vi "AlliGator Lifetime & Other Parameters Panel.vi"() -> ()   [LabVIEW 2021, in "AlliGator Lifetime & Other Parameters.lvlib"]
uses:
  AlliGator Lifetime & Other Parameters.lvlib
  AlliGator Lifetime & Other Parameters Ctrl Refnums.ctl
  Globals, Variables, Constants/AlliGator Refnums List.ctl
  Settings/AlliGator Settings List.ctl
  Graphs/XY Graph/XY Graph Event.ctl
  <vilib>/Utility/miscctls.llb/LVPoint32TypeDef.ctl
  Action Engine/AlliGator Q Element.ctl
  Action Engine/AlliGator Q Event.ctl
  Graphs/XY Graph/New Plot Information.ctl
  Graphs/Plot Scales.ctl
  Graphs/LabVIEW Plot Interpolation.ctl
  Graphs/Plot Point Style.ctl
  Graphs/XY Graph/XY Graph Mouse Click Event Data.ctl
  Graphs/XY Graph/XY Graph Refnum.ctl
  Variant/Variant to Data/Variant to Boolean.vi
  Settings/AlliGator Settings+.lvlib
  Variant/Variant to Data/Variant to Data.lvlib
  Notebook/Notebook.lvlib
  Action Engine/AlliGator Action Engine.lvlib
  GUI/GUI.lvlib
  GUI/AlliGator GUI.lvlib
  Error/Error.lvlib
  Graphs/XY Graph/XY Graph Add-Ons.lvlib
  Python Plugins API/AlliGator Python Plugins.lvlib
  Decay Analysis/Decay Processing/AlliGator Decay Processing.lvlib
  Graphs/Graphs.lvlib
  Phasor Ratio/AlliGator Phasor Ratio.lvlib
  Utilities/Utilities.lvlib
panel:
  in  "Pin Button":bool=TRUE
  out "Lifetime & Other Parameters Graph TipStrip":string caption="Lifetime Graph TipStrip"
  out "Lifetime & Other Parameters Graph":cluster{"X Array":dbl[], "Y Array":dbl[]}[](graph)
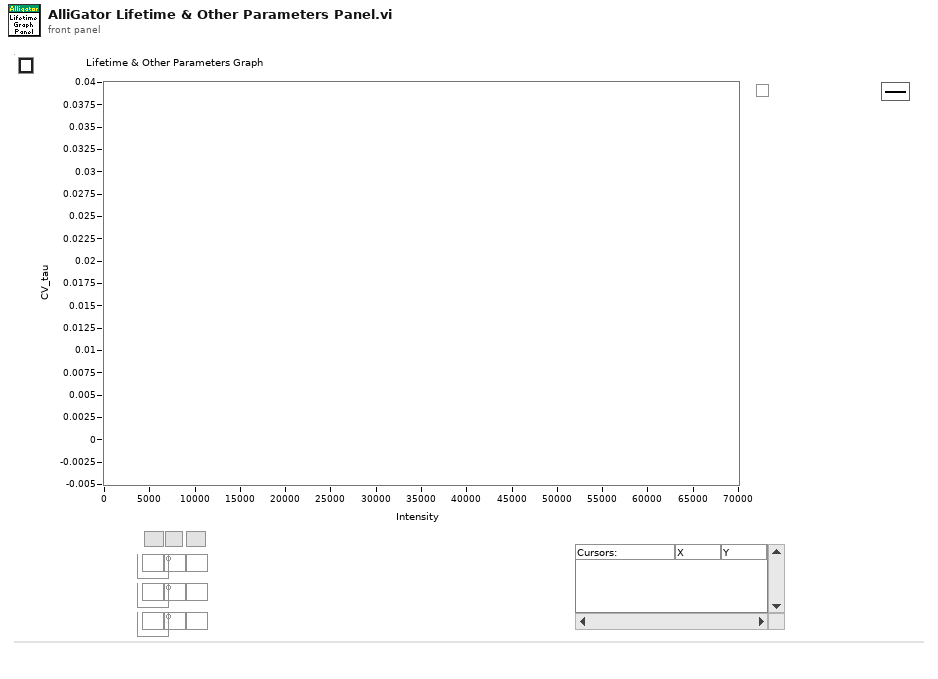
[diagram p1: front panel]
types:
  T1 = typedef "AlliGator GUI.lvlib/AlliGator Refnums List.ctl" = enum16{"---------- AlliGator Control Refnums ----------", "AlliGator Tab Control Refnum", "Dataset Ctrl Refnums", "Image Histogram Ctrl Refnums", "Intensity Time Trace Ctrl Refnums", "Decay Graph Ctrl Refnums", "Decay Statistics Graph Ctrl Refnums", "Phasor Graph Ctrl Refnums", "Phasor Ratio Graph Ctrl Refnums", "Phasor Plot Ctrl Refnums", "Lifetime & Other Parameters Ctrl Refnums", "Decay Fit Parameter Map Ctrl Refnums", "Parameter Map Ctrl Refnums", "Other AlliGator Ctrl Refnums", "---------- AlliGator Menu Refnums ----------", "AlliGator Menu", "---------- IO Device ID ----------", "Mouse ID", "Keyboard ID"}
  T2 = typedef "AlliGator Lifetime & Other Parameters.lvlib/AlliGator Lifetime & Other Parameters Ctrl Refnums.ctl" = cluster{"Lifetime Graph":refnum<vi>}
  T3 = cluster{"Event Registration Refnum":refnum<event-registration>, "Event Registration Refnum":refnum<event-registration>}
  T4 = typedef "AlliGator Settings+.lvlib/AlliGator Settings List.ctl" = enum16{"GUI:Visible Settings Tab", "GUI:Last Run Version", "Source Image:Use Image Histogram for Contrast", "Source Image:Low Count Pixels Rejection Options", "Source Image:High Count Pixels Rejection Options", "Source Image:Use Image Brightness", "Source Image:Blend Overlay with Image Background", "Source Image:Use Fixed ROI Diameter", "Source Image:ROI Diameter", "Source Image:ROI Center Color", "Source Image:Peak Threshold", "Source Image:Intensity Threshold", "Source Image:Image Binning Options", "Source Image:Image Smoothing Options", "Source Image:Image Histogram Active", "Source Image:Invert Binary Mask", "Source Image:Hot Pixel Removal", "Source Image:Overlay Analyzed ROI Center", "Source Image:Auto-Adjust Contrast", "Source Image:Histogram Lower Percentile", "Source Image:Histogram Upper Percentile", "Source Image:Lock ROI with Maps", "Source Image:Save Source Image", "Source Image:Scale Bar Options", "Source Image:Image Resolution (Pixel Size)", "Source Image:Flatfield Correction", "Source Image:Show Dead Left Columns Correction", "Source Image:Dead Left Columns Correction", "Source Image:Image Pre-Processing Operations Order", "Source Image:Overlay ROI Median", "Source Image:Median Overlay Color", "Data Information:Gate Width", "Data Information:Nanotime Gate Separation", "Data Information:Macrotime Gate Separation", "Data Information:Gate Step", "Data Information:# Gates", "Data Information:Gate Image Exposure", "Data Information:Gate Image Integration", "Data Information:Gates to Skip", "Data Information:Gates to Keep", "Data Information:Define Gates to", "Data Information:Channel Name", "Data Information:Available Channel Names", "Data Information:Channel Arithmetic", "Data Information:Background File Subtraction", "Data Information:Background File", "Data Information:Background Scaling Factor", "Data Information:Background Pile-up Correction", "Data Information:Background Pixel Well Capacity", "Data Information:Laser Period", "Data Information:SYNC Period", "Data Information:Pile-up Correction", "Data Information:Pixel Well Capacity", "Data Information:Dataset Scaling Factor", "Fluorescence Decay_Decay Pre-Processing:Reverse Gates", "Fluorescence Decay_Decay Pre-Processing:Verbose Decay Pre-Processing", "Fluorescence Decay_Decay Pre-Processing:Use Decay Pre-Processing", "Fluorescence Decay_Decay Pre-Processing:Background Subtraction", "Fluorescence Decay_Decay Pre-Processing:Background Definition Range", "Fluorescence Decay_Decay Pre-Processing:Baseline Subtraction Method", "Fluorescence Decay_Decay Pre-Processing:Decay Pre-Processing Operations Order", "Fluorescence Decay_Decay Pre-Processing:Smoothing Parameter", "Fluorescence Decay_Decay Pre-Processing:Shift Decay", "Fluorescence Decay_Decay Pre-Processing:Decay Shift Parameters", "Fluorescence Decay_Decay Pre-Processing:Fold Decay", "Fluorescence Decay_Decay Pre-Processing:# Folds", "Fluorescence Decay_Decay Pre-Processing:1-Normalize Decay", "Fluorescence Decay_Decay Pre-Processing:[0-1]-Normalize Decay", "Fluorescence Decay_Decay Pre-Processing:Smoothen Decay", "Fluorescence Decay_Decay Pre-Processing:Extrapolate Decay", "Fluorescence Decay_Decay Pre-Processing:Use Periodicity", "Fluorescence Decay_Decay Pre-Processing:Use Cursors", "Fluorescence Decay_Decay Pre-Processing:Tail Fraction", "Fluorescence Decay_Decay Pre-Processing:Head Fraction", "Fluorescence Decay_Decay Pre-Processing:Additional Points", "Fluorescence Decay_Decay Pre-Processing:Straighten Decay", "Fluorescence Decay_Decay Pre-Processing:Constant Background", "Fluorescence Decay_Decay Pre-Processing:Pixel-Normalize Decay", "Fluorescence Decay_Advanced Analysis:Extract IRF instead of Decay", "Fluorescence Decay_Advanced Analysis:IRF Extraction Options", "Fluorescence Decay_Advanced Analysis:IRF Optimization Options", "Fluorescence Decay_Advanced Analysis:Square Pulse Options", "Fluorescence Decay_Advanced Analysis:IRF Order", "Fluorescence Decay_Advanced Analysis:IRF Time Constants", "Fluorescence Decay_Advanced Analysis:Wavelet Analysis Options", "Fluorescence Decay_Advanced Analysis:Average Lifetime Options", "Fluorescence Decay_Fit Options:Fit Options", "Fluorescence Decay_Fit Options:Use Legacy Fitting Approach", "Fluorescence Decay_Fit Options:Use Data Information Laser Period", "Fluorescence Decay_Fit Parameters:Displayed Fit Parameters", "Fluorescence Decay_Fit Parameters:Fit Parameter Constraints", "Fluorescence Decay_Fit Parameters:Export Tabulated Results", "Fluorescence Decay_Fit Parameters:MLE Baseline Offset Type", "Fluorescence Decay_Fit Parameters:MLE Baseline Offset", "Fluorescence Decay_Fit Parameters:Guess Parameter Names", "Fluorescence Decay_Fit Parameters:Guess Parameter Values", "Fluorescence Decay_Fit Parameters:Guess Parameters Options", "Fluorescence Decay_Fit Parameters:Optimal Offset Selection Criterion", "Fluorescence Decay_Styles:Show Last Decay Only", "Fluorescence Decay_Styles:Decay Graph Color Array", "Fluorescence Decay:Decay Graph Active", "Fluorescence Decay Statistics:Min Peak Value", "Fluorescence Decay Statistics:Reject Low Decay Peak Pixels", "Fluorescence Decay Statistics:Reject High Decay Peak Pixels", "Fluorescence Decay Statistics:Max Peak Value", "Time Traces:Use File Timestamp", "Time Traces:Time Step", "Time Traces:Use Intensity Correction File", "Time Traces:Intensity Correction File", "Phasor Plot:Phasor Plot Smoothing Options", "Phasor Plot:Phasor Plot Size", "Phasor Plot:Phasor Plot Graphics Options", "Phasor Plot:Cumulative Phasor Plot", "Phasor Plot:Use Phasor Brightness", "Phasor Plot:Blend Overlay with Phasor Background", "Phasor Plot:Save Phasor Plot", "Phasor Plot:Show References", "Phasor Plot:Phasor Ratio Decay Range", "Phasor Plot:Exponential Fading", "Phasor Plot:Phasor Ratio Reference Colors", "Phasor Plot:Reference Radius", "Phasor Plot:Show Color Map Vertices", "Phasor Plot:Phasor Plot Active", "Phasor Plot:Phasor Ratio Color Map Type", "Phasor Plot:Phasor Ratio Color Map", "Phasor Plot:Phasor Ratio Display Range", "Phasor Plot:Selected Image ROI(s)", "Phasor Plot:All Image ROIs", "Phasor Plot:Selected Phasor Plot ROI(s)", "Phasor Plot:All Phasor Plot ROIs", "Phasor Plot:Phasor Ratio Color-Coded Quantity", "Phasor Plot:Store Phasor Harmonics", "Phasor Plot:Draw Reference Segment", "Phasor Plot:User-Defined Quantity", "Phasor Plot:Color Scale High Color", "Phasor Plot:Color Scale Low Color", "Phasor Plot:Intensity-weighted Phasor Plot", "Phasor Graph:Phasor Frequency", "Phasor Graph:Phasor Ratio Type", "Phasor Graph:Pixel-level Phasor Computation", "Phasor Graph:Save Phasor Graph", "Phasor Graph:Phasor Graph Active", "Phasor Graph:Phasor SDV Options", "Phasor Graph:Intensity-weighted Phasor Graph", "Phasor Graph:Define Shortest Lifetime as", "Phasor Calibration:Use Backup Calibration if needed", "Phasor Calibration:Backup Calibration Type", "Phasor Calibration:Calibration Type", "Phasor Calibration:Calibration Lifetime", "Phasor Calibration:Calibration Map Algorithm", "Single-Exponential Phasor Locus (SEPL):Gate Parameters", "Single-Exponential Phasor Locus (SEPL):User-defined Gate", "Single-Exponential Phasor Locus (SEPL):User-defined IRF", "Single-Exponential Phasor Locus (SEPL):Phasor Parameters", "Single-Exponential Phasor Locus (SEPL):Decay & IRF Parameters", "Single-Exponential Phasor Locus (SEPL):Display Parameters", "Lifetime Analysis:Decay Analysis Parameters", "Lifetime Analysis:Lifetime Map Active", "Plugins:Python Settings", "Miscellaneous:Verbose Mode", "Miscellaneous:Beep after Script", "Miscellaneous:Saved Image File Format", "Miscellaneous:Exported Gate Image Settings", "Miscellaneous:Include Loading in Timing", "Miscellaneous:Verbose Settings Mode", "Miscellaneous:Histogram Options", "Miscellaneous:Beep on Error", "Miscellaneous:# Logical Processors Used", "Miscellaneous:ROI Description Max Characters", "Miscellaneous:Verbose Error Mode", "Miscellaneous:Transparent Mask Color"}
  T5 = typedef "AlliGator Action Engine.lvlib/AlliGator Q Element.ctl" = cluster{"AlliGator Q Event":T6, "Data":variant}
  T6 = typedef "AlliGator Action Engine.lvlib/AlliGator Q Event.ctl" = enum16{"---- Files ----", "Files:Set Batch Export Files To Save", "Files:Set Dataset Loading & Pre-processing Options", "Files:Check #Frames in Dataset", "Files:Increment Frame Index", "Files:Open Mask Image", "Files:Open White Light Image", "Files:Open Single Dataset", "Files:New Folder of Folders Selected", "Files:Load File (all Types)_Scriptable", "Files:Move Flattened Series to Folders Series", "Files:Select Folder", "Files:Load FLI Dataset", "Files:Load Swiss SPAD 1 Dataset", "Files:Load Swiss SPAD 2 Dataset", "Files:Load .sdt FLI Dataset", "Files:Load .ptu FLI Dataset", "Files:Load .bin FLI Dataset", "Files:Load Single Gate Image Folder", "Files:Load I/m/phi Dataset (deprecated)", "Files:Load Single Image", "Files:Subtract Background File", "Files:Export FLI Dataset", "Files:Load HDF5 FLI Dataset", "Files:Set Destination File Path", "Files:Save Mask Image", "Files:Batch Conversion", "Files:New Folder Selected", "Files:Close FLI Dataset", "Files:Close FLI Dataset Series", "Files:Close White Light Image", "Files:Close Mask Image", "---- FLI Dataset ----", "FLI Dataset:Channel Arithmetic", "FLI Dataset:Export Average Lifetime Map as ASCII", "FLI Dataset:Export User-Defined Quantity Map as ASCII", "FLI Dataset:Python Function FLI Dataset Event", "FLI Dataset:ROI Analysis", "FLI Dataset:Tilted Logistic Square Gated IRF Characteristics Map", "FLI Dataset:Logistic Square Gated IRF Characteristics Map", "FLI Dataset:Square Gated IRF Characteristics Map", "FLI Dataset:Multi-ROI Single-Pixel Phasor Analysis", "FLI Dataset:Multi-ROI Single-Pixel NLSF Analysis", "FLI Dataset:All ROIs IRF Extraction", "FLI Dataset:All ROIs Decay Fit Non-Interactive (Fast + Individual IRF)", "FLI Dataset:All ROIs Phasor Analysis", "FLI Dataset:All ROIs Decay Fit", "FLI Dataset:Fluorescence Decay Statistics", "FLI Dataset:Update Decay Statistics Graph", "FLI Dataset:Get Decay from ROI", "FLI Dataset:All ROIs Average Lifetimes", "FLI Dataset:Save/Load Local IRFs", "FLI Dataset:Clear Local IRFs", "FLI Dataset:Phasor Calibration Maps (# Gates Series) Script", "FLI Dataset:Calibrated Phasor Map Series", "---- FLI Dataset Series ----", "FLI Dataset Series:Sum All Datasets in Series", "FLI Dataset Series:Add Dataset to Accumulated Dataset", "FLI Dataset Series:Display Accumulated Dataset", "FLI Dataset Series:Clear Dataset Series Sum", "FLI Dataset Series:Time-Series Analysis (NLSF)", "FLI Dataset Series:Time-Series Analysis (Phasor)", "---- Image ----", "Image:Update Image Profile Plots", "Image:Image Histogram Cursor Move", "Image:Image Histogram", "Image:Image Contrast", "Image:Set Image Histogram Cursor Move Flag", "Image:Clear Image Overlay", "Image:Use ROI as Search Area", "Image:Set ROI Diameter", "Image:Save Image Data as TIFF", "Image:Save Displayed Image with Overlay", "Image:Save Image Overlay Only", "Image:Save Image as Hot Pixel Mask", "Image:Change Source Image Color Palette", "Image:Copy Image to Clipboard", "Image:Source Image ROI Selection", "Image:Delete All ROIs", "Image:Delete All Unselected ROIs", "Image:Delete ROI", "Image:Merge All ROIs", "Image:Store ROI", "Image:Source Image ROI Storage", "Image:Export ROI Description to Notebook", "Image:Save ROI", "Image:Load ROI", "Image:Paste ROI Definition", "Image:Clear ROI", "Image:Identify ROIs in Mask Image", "Image:Create Complementary ROI", "Image:Create Contour ROI", "Image:Create ROI(s) from Pixels with Peak above Min_Scriptable", "Image:Create ROI(s) from Pixels with Intensity above Min_Scriptable", "Image:Compute ROI Statistics", "Image:Delete ROI(s) based on ROI Characteristics", "Image:Create ROI Grid", "Image:ROI to Individual Pixel ROIs", "Image:Python Function Source Image Event", "Image:Show Phasor Calibration Map ROI Centers", "Image:Convert ROI to Mask Image", "Image:Mouse Move", "Image:Mouse Up", "Image:Set Source Image Mouse Move Flag", "Image:Add Scale Bar Overlay", "Image:Delete Existing ROIs Option", "Image:Overlay ROI Median", "Image:Check Current ROI", "Image:Update True Pixel Value", "Image:Use ROI", "---- Decay ----", "Decay:Clear IRF/Reference Plot", "Decay:Add Decay to Graph", "Decay:Smoothen Plot", "Decay:Smoothen Plot Tail", "Decay:Average Selected Plots", "Decay:Extract IRF", "Decay:Optimal IRF Extraction", "Decay:Threshold IRF", "Decay:Fit to Model IRF", "Decay:Fit IRF to Square Gate", "Decay:Fit IRF to Logistic Square Gate", "Decay:Fit IRF to Tilted Logistic Square Gate", "Decay:Create Bounding Cursors Set", "Decay:Export Bounding Cursors Definition to Notebook", "Decay:Denoise Plot", "Decay:Compute Cumulative Function", "Decay:Use as Reference Decay", "Decay:Show Reference Decay/IRF", "Decay:Extrapolate Decay", "Decay:Create Head & Tail Bounding Cursors", "Decay:Store Cursor-defined Head & Tail Fractions", "Decay:Rebin Plot", "Decay:1-Normalize Decay", "Decay:[0-1]-Normalize Plot", "Decay:Straighten Decay", "Decay:Shift Decay", "Decay:Fold Decay", "Decay:Fit Decay", "Decay:Global Fit of Selected Decays", "Decay:Post Global Fit Script", "Decay:Add Global Fit Parameters to Graph", "Decay:Add Decay Parameter(s) to Plot (Graph)", "Decay:Export Decay to Phasor Graph", "Decay:Compute Average Lifetime", "Decay:Plot Convolution", "Decay:Graph Tip Strip Update", "---- Decay Statistics ----", "Decay Statistics:Tip Strip Update", "---- Intensity Time Trace ----", "Intensity Time Trace:Use File Timestamp", "Intensity Time Trace:Load Intensity Corrections File", "Intensity Time Trace:Clear Intensity Corrections File", "Intensity Time Trace:Tip Strip Update", "---- Phasor Plot ----", "Phasor Plot:Build Phasor Plot", "Phasor Plot:Change Phasor Plot Color Palette", "Phasor Plot:Adjust Phasor Plot Display Range", "Phasor Plot:Highlight Image ROI in Phasor Plot", "Phasor Plot:Save Phasor Plot Image with Overlay", "Phasor Plot:Export Complex Phasor Map", "Phasor Plot:Export Phasor Ratio Map", "Phasor Plot:Export Average Lifetime Map", "Phasor Plot:Compute Phase Lifetime Histogram", "Phasor Plot:Compute Phasor Ratio Histogram", "Phasor Plot:Compute Phase Lifetime vs Intensity Scatter Plot", "Phasor Plot:Weber 2-Component Decomposition", "Phasor Plot:Update Phasor Color Map Vertices", "Phasor Plot:Clear Phasor Overlay", "Phasor Plot:Use Segment Extremities as References", "Phasor Plot:Use UC/Segment Intersections as References", "Phasor Plot:Use UC/Principal Axis Intersections as References", "Phasor Plot:Use UC/Linear Fit Intersections as References", "Phasor Plot:Update Phasor Plot Reference", "Phasor Plot:Show Local Phasor Info in Phasor Plot", "Phasor Plot:Update Phasor Plot State", "Phasor Plot:Phasor Plot ROI Storage", "Phasor Plot:Phasor Plot ROI Selection", "Phasor Plot:Python Function Phasor Plot Event", "Phasor Plot:Overlay Phasor ROI, Ratio or Map in Source Image", "Phasor Plot:Compute Decay of Selected Phasors", "Phasor Plot:Phasor at Image Pixel", "Phasor Plot:Mouse Move", "Phasor Plot:Mouse Up", "Phasor Plot:Display Range Mouse Move", "Phasor Plot:Set Mouse Move Flag", "Phasor Plot:Update True Phasor Plot Value", "---- Phasor Graph ----", "Phasor Graph:Get Phasor Value", "Phasor Graph:Create New Phasor Plot Dialog", "Phasor Graph:Update Last Phasor Value", "Phasor Graph:Update Phasor (m, phi)", "Phasor Graph:Remove Single Phasor from Plot", "Phasor Graph:Add Single Phasor to Plot", "Phasor Graph:Remove Phasor Plot", "Phasor Graph:Remove Selected Phasor Plots", "Phasor Graph:Clear Phasor Data", "Phasor Graph:Clear Phasor Graph", "Phasor Graph:Cursor Move", "Phasor Graph:Draw Cursor Connecting Line", "Phasor Graph:Clear Cursor Connecting Line", "Phasor Graph:Find UC Intersection", "Phasor Graph:Use UC/Cursor-Defined Line Intersections", "Phasor Graph:Use Selected Plots Fitted Line/UC Intersections", "Phasor Graph:Use Selected Plots Principal Axis/UC Intersections", "Phasor Graph:Show Single Phasor", "Phasor Graph:Save Single Phasor Plot", "Phasor Graph:Save All Phasor Plots", "Phasor Graph:Load Phasor Plot(s)", "Phasor Graph:Phasor Multiplication", "Phasor Graph:Compute Average Phasor", "Phasor Graph:Compute Multiple Average Phasors (Selected Plots)", "Phasor Graph:Export Single Phasor Plot Phase Lifetimes", "Phasor Graph:Parameter 2 vs Parameter 1 Scatter Plot", "Phasor Graph:Use Cursor n Location", "Phasor Graph:Set Reference n to Current Phase Lifetime Value", "Phasor Graph:Set Reference n to Lifetime Value", "Phasor Graph:Set Cursor n Location", "Phasor Graph:Save Phasor Graph Image", "Phasor Graph:Update SEPL Plot", "Phasor Graph:Export Single Phasor Plot Data", "Phasor Graph:Export Selected Phasor Plots Data", "Phasor Graph:Python Function Phasor Graph Event", "Phasor Graph:Tip Strip Update", "---- Calibration ----", "Calibration:Set Calibration Type", "Calibration:Load/Save Phasor Calibration", "Calibration:Load/Save Phasor Calibration Series", "Calibration:Load/Save Phasor Calibration Map", "Calibration:Use as Calibration", "Calibration:Compute Optimal Calibration from Phasor References", "Calibration:Clear Phasor Calibration", "Calibration:Single Phasor Calibration Information", "Calibration:Use as Calibration Series", "Calibration:Use as Calibration Map", "Calibration:Clear Calibration Series", "Calibration:Phasor Calibration Series Information", "Calibration:Clear Calibration Map", "Calibration:Phasor Calibration Map Information", "Calibration:Apply Phasor Calibration", "Calibration:Update Single Plot Calibration", "Calibration:Update Multiple Plots Calibration", "Calibration:Clear Single Plot Calibration", "Calibration:Clear All Plots Calibrations", "Calibration:Clear Plot(s) Calibration(s)?", "---- Phasor Ratio ----", "Phasor Ratio:Clear Reference n", "Phasor Ratio:Toggle Selected Plot(s)  Lock to Reference 1", "Phasor Ratio:Use as Reference n", "Phasor Ratio:Send Reference n to Notebook", "Phasor Ratio:Toggle Selected Plot(s)  Lock to Reference 2", "Phasor Ratio:Compute Phasor Ratio at Mouse Location", "Phasor Ratio:Compute Phasor Plot's Average Phasor Ratio", "Phasor Ratio:Compute Time-Series Phasor Ratios", "Phasor Ratio:Fit Line to Phasor Ratio Plot", "Phasor Ratio:Save References", "Phasor Ratio:Load References", "Phasor Ratio:Update Phasor Reference 1", "Phasor Ratio:Update Phasor Reference 2", "Phasor Ratio:Move Cursor n to Reference n", "Phasor Ratio:Use as Phasor Reference 1 Lifetime", "Phasor Ratio:Use as Phasor Reference 2 Lifetime", "Phasor Ratio:Export Phasor Ratio Map as ASCII", "Phasor Ratio:Tip Strip Update", "---- Lifetime & Other Parameters Graph ----", "Lifetime:Compute Sliced Mean, SDV and CV Plots", "Lifetime:Plot Decay Shifts", "Lifetime:Plot Histogram", "---- Decay Fit Parameter Map ----", "Decay Fit Parameter Map:Export ROI NLSF Data as ASCII", "Decay Fit Parameter Map:Set Decay Fit Parameter Map Selection", "Decay Fit Parameter Map:Build Decay Fit Parameter Map", "Decay Fit Parameter Map:Change Decay Fit Parameter Map Color Palette", "Decay Fit Parameter Map:Export Decay Fit Parameter Map Data as ASCII", "Decay Fit Parameter Map:Export All Decay Fit Parameter Maps Data as ASCII", "Decay Fit Parameter Map:Selected Parameter Scatterplot", "Decay Fit Parameter Map:Parameter 2 vs Parameter 1 Scatterplot", "Decay Fit Parameter Map:Save Decay Fit Parameter Map Image", "Decay Fit Parameter Map:Save-Load IRFs & Fit Data", "Decay Fit Parameter Map:Update Local Decay Plots", "Decay Fit Parameter Map:Python Function Decay Fit Parameters Map Event", "Decay Fit Parameter Map:Overlay Decay Fit Parameter Map in Source Image", "Decay Fit Parameter Map:Selected Parameter vs Intensity Scatterplot", "Decay Fit Parameter Map:Mouse Up", "Decay Fit Parameter Map:Mouse Move", "Decay Fit Parameter Map:Display Range Mouse Move", "Decay Fit Parameter Map:Change Map Resolution", "Decay Fit Parameter Map:Variance Significance Maps", "Decay Fit Parameter Map:Fit Result Constraints Window", "Decay Fit Parameter Map:Use ROI", "---- Parameter Map ----", "Parameter Map:Export ROI Parameters Data as ASCII", "Parameter Map:Add Parameter Map Set", "Parameter Map:Delete Parameter Map Set", "Parameter Map:Update Parameter List", "Parameter Map:Build Parameter Map", "Parameter Map:Change Parameter Map Color Palette", "Parameter Map:Export Parameter Map Data as ASCII", "Parameter Map:Export All Parameter Maps Data as ASCII", "Parameter Map:Selected Parameter Scatterplot", "Parameter Map:Parameter 2 vs Parameter 1 Scatterplot", "Parameter Map:Selected Parameter vs Intensity Scatterplot", "Parameter Map:Save Parameter Map Image", "Parameter Map:Save-Load IRFs & Parameter Maps (TODO)", "Parameter Map:Set Parameter Map Selection", "Parameter Map:Python Function Parameter Map Event", "Parameter Map:Overlay Parameter Map in Source Image", "Parameter Map:Update Local Decay Plots", "Parameter Map:Mouse Up", "Parameter Map:Mouse Move", "Parameter Map:Display Range Mouse Move", "Parameter Map:Use ROI", "---- Generic Graph ----", "Generic Graph:Generic XY Graph Event", "Generic Graph:Python Function XY Graph Event", "Generic Graph:New Plot", "Generic Graph:Save Plot", "Generic Graph:XY Plot Histogram", "Generic Graph:Set XY Graph Plot Name", "Generic Graph:Set Last Cursor Style", "Generic Graph:Tip Strip Update", "---- GUI ----", "GUI:Start Script", "GUI:Type of Displayed Image Changed", "GUI:Gate Image Slide Changed", "GUI:Show Busy Icon", "GUI:Show Busy Icon & Abort Button", "GUI:Hide Busy Icon", "GUI:Hide Busy Icon & Abort Button", "GUI:Abort", "GUI:End Script", "GUI:Start Timing", "GUI:End Timing", "GUI:Set State Indicator", "GUI:Send Parameters JSON Strings to Clipboard", "GUI:Set Gate Step", "GUI:Idle", "GUI:Initialization", "GUI:Quit", "GUI:Increment Dataset Index", "GUI:Set Dataset Index to -1", "GUI:Time Series Slider Moved", "GUI:Time Series Slider Changed", "GUI:Toggle Playback or Loop", "GUI:Playback Script", "GUI:Set Phasor Frequency", "GUI:Open Window", "GUI:Start Test Script", "GUI:End Test Script", "GUI:Set Verbose Mode", "GUI:Set Verbose Settings Mode", "GUI:Initialize Python Session", "DEBUG"}
  T7 = typedef "XY Graph Add-Ons.lvlib/XY Graph Event.ctl" = cluster{"Item Tag":string, "XY Graph Refnum":refnum<vi>, "Coords":T8, "Item Path":string}
  T8 = typedef "LVPoint32TypeDef.ctl" = cluster{"Horizontal":i32, "Vertical":i32}
  T9 = typedef "XY Graph Add-Ons.lvlib/XY Graph Mouse Click Event Data.ctl" = cluster{"Multiplot XY Graph":T10, "Mouse Coordinates":T8}
  T10 = typedef "XY Graph Add-Ons.lvlib/XY Graph Refnum.ctl" = refnum<vi>
  T11 = typedef "XY Graph Add-Ons.lvlib/New Plot Information.ctl" = cluster{"Multiplot XY Graph":refnum<vi>, "Plot Name":string, "Plot Scales":T12, "Plot Interpolation":T13, "Point Style":T14, "Plot Color":u32, "Plot Metadata":variant}
  T12 = typedef "XY Graph Add-Ons.lvlib/Plot Scales.ctl" = cluster{"X Scale":u32, "Y Scale":u32}
  T13 = typedef "Graphs.lvlib/LabVIEW Plot Interpolation.ctl" = enum16{"Point (.)", "Stepwise Right (--.)", "Line + Point (\\. /)", "Stepwise Left (.--)", "Stepwise Centered (-.-)", "Stepwise Vertical (|.|)", "Line (-)", "Use Previous Plot's Style"}
  T14 = typedef "Graphs.lvlib/Plot Point Style.ctl" = enum16{"not defined", "None", "Empty Circle", "Filled Circle", "Thick Circle", "Dotted Circle", "Empty Square", "Filled Square", "Thick Square", "Dotted Square", "Small Filled Square", "Dot", "Cross", "Tiny Cross", "Large X", "Small x", "Diamond", "Small Empty Square"}
  T15 = typedef "AlliGator Phasor Ratio.lvlib/AlliGator Phasor Ratio Graph Ctrl Refnums.ctl" = cluster{"Phasor Ratio Graph":refnum<vi>}
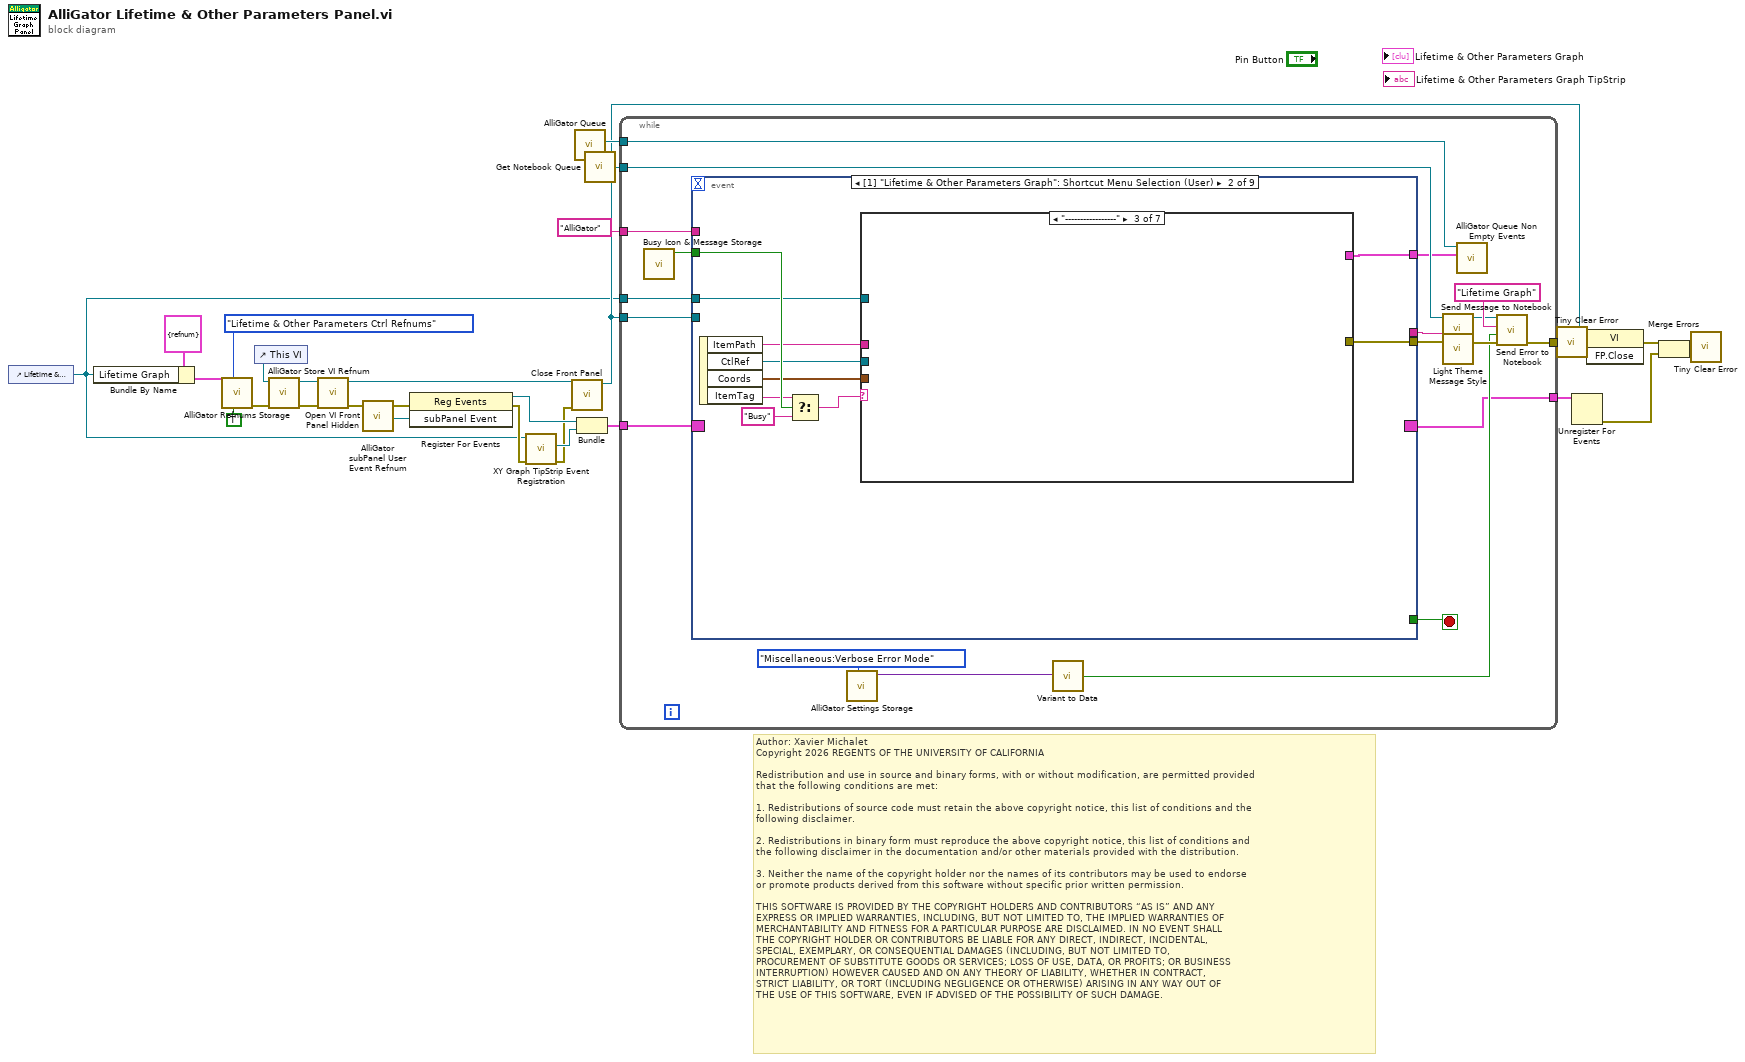
[diagram p0: block diagram]
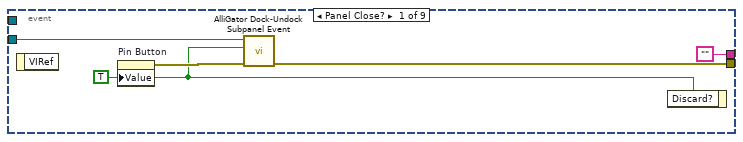
[diagram p2: hidden frame]
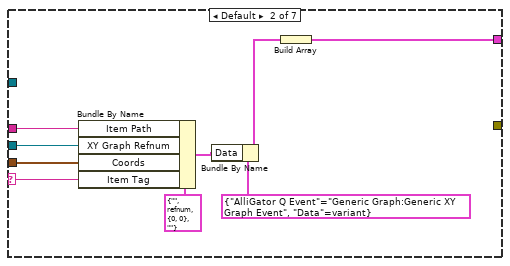
[diagram p4: hidden frame]
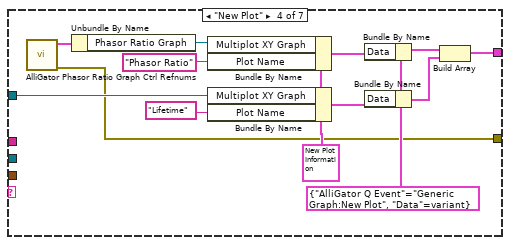
[diagram p5: hidden frame]
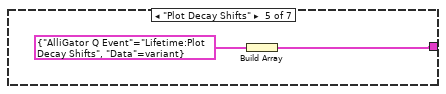
[diagram p6: hidden frame]
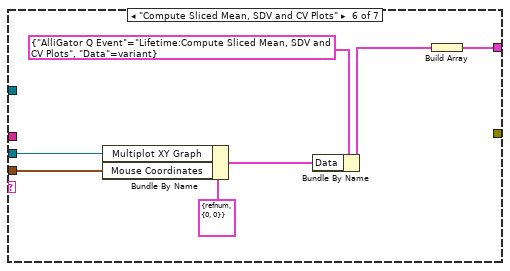
[diagram p7: hidden frame]
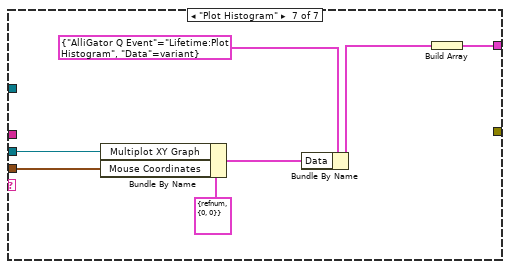
[diagram p8: hidden frame]
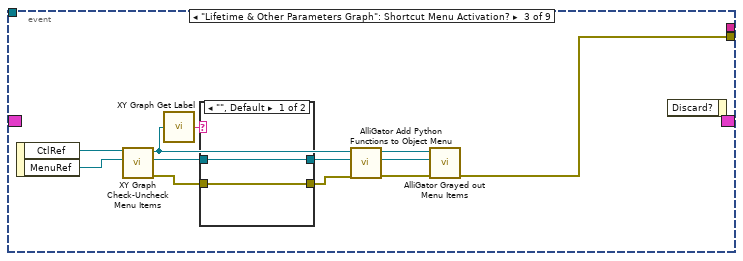
[diagram p9: hidden frame]
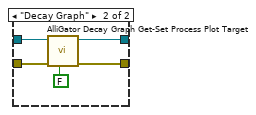
[diagram p10: hidden frame]
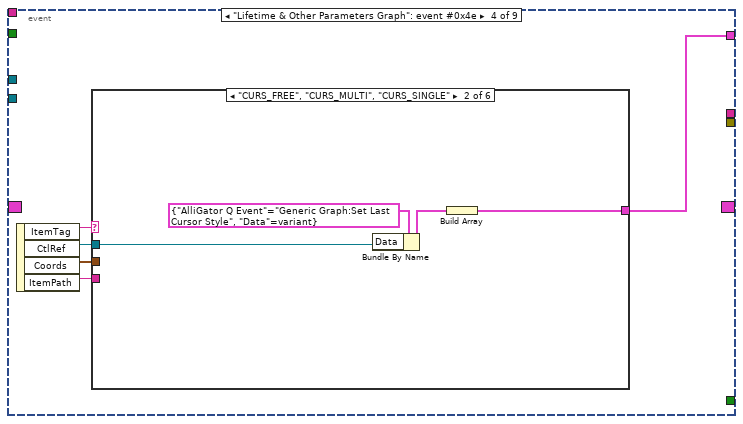
[diagram p11: hidden frame]
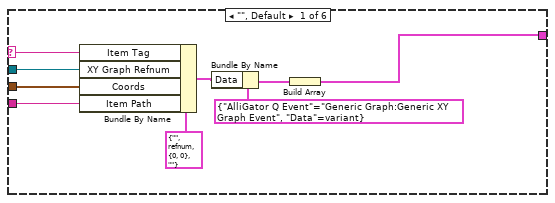
[diagram p12: hidden frame]
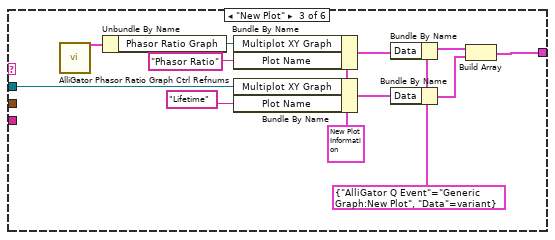
[diagram p13: hidden frame]
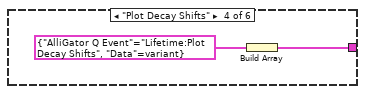
[diagram p14: hidden frame]
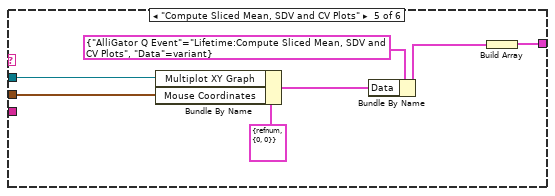
[diagram p15: hidden frame]
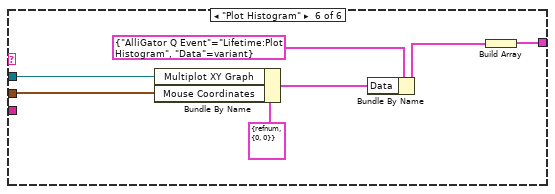
[diagram p16: hidden frame]
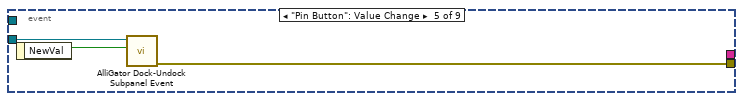
[diagram p17: hidden frame]
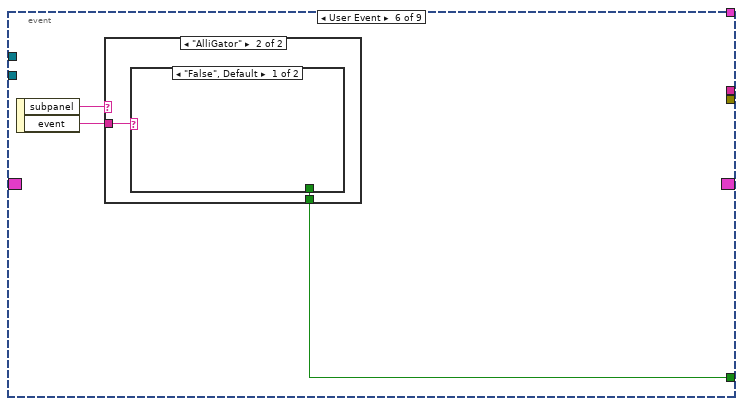
[diagram p18: hidden frame]
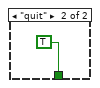
[diagram p20: hidden frame]
diagram:
  # "Author: Xavier Michalet\nCopyright 2026 REGENTS OF THE UNIVERSITY OF CALIFORNIA\n\nRedistribution and use in source and binary forms, with or without modification, are permitted provided\nthat the following conditions are met:\n\n1. Redistributions of source code must retain the above copyright notice, this list of conditions and the\nfollowing disclaimer.\n\n2. Redistributions in binary form must reproduce the above copyright notice, this list of conditions and\nthe following disclaimer in the documentation and/or other materials provided with the distribution.\n\n3. Neither the name of the copyright holder nor the names of its contributors may be used to endorse \nor promote products derived from this software without specific prior written permission.\n\nTHIS SOFTWARE IS PROVIDED BY THE COPYRIGHT HOLDERS AND CONTRIBUTORS “AS IS” AND ANY \nEXPRESS OR IMPLIED WARRANTIES, INCLUDING, BUT NOT LIMITED TO, THE IMPLIED WARRANTIES OF\nMERCHANTABILITY AND FITNESS FOR A PARTICULAR PURPOSE ARE DISCLAIMED. IN NO EVENT SHALL\nTHE COPYRIGHT HOLDER OR CONTRIBUTORS BE LIABLE FOR ANY DIRECT, INDIRECT, INCIDENTAL, \nSPECIAL, EXEMPLARY, OR CONSEQUENTIAL DAMAGES (INCLUDING, BUT NOT LIMITED TO, \nPROCUREMENT OF SUBSTITUTE GOODS OR SERVICES; LOSS OF USE, DATA, OR PROFITS; OR BUSINESS\nINTERRUPTION) HOWEVER CAUSED AND ON ANY THEORY OF LIABILITY, WHETHER IN CONTRACT, \nSTRICT LIABILITY, OR TORT (INCLUDING NEGLIGENCE OR OTHERWISE) ARISING IN ANY WAY OUT OF\nTHE USE OF THIS SOFTWARE, EVEN IF ADVISED OF THE POSSIBILITY OF SUCH DAMAGE."
  n1 = control-ref of="Lifetime & Other Parameters Graph"() -> (w5:refnum<vi>)
  n2 = Bundle By Name(cluster=T2 {"Lifetime Graph"=refnum} ("Lifetime & Other Parameters Graph Ctrl Refnums"), "Lifetime Graph"=w5) -> (w16:T2)
  n3 = call "AlliGator Refnums Storage.vi"("Get(F)/Set"=TRUE, "AlliGator Refnum List"=AlliGator_Refnums_List."Lifetime & Other Parameters Ctrl Refnums", "Data in"=w16) -> ("Error Out"=w4:errorcluster)  [unwired: 7 in, 1 out]
  n4 = control-ref of="This VI"() -> (w2:refnum<vi>)
  n5 = call "AlliGator Store VI Refnum.vi"("error in (no error)"=w4, "VI Refnum"=w2) -> ("error out"=w3:errorcluster, "VI Refnum (dup)"=w1:refnum<vi>)  [unwired: 7 in, 1 out]
  n6 = call "Open VI Front Panel Hidden.vi"("error in"=w3, "VI in"=w1) -> ("error out"=w10:errorcluster, "VI out"=w7:refnum<vi>)  [unwired: 8 in]
  n7 = call "AlliGator subPanel User Event Refnum.vi"() -> ("subPanel Event"=w24:refnum<user-event>)  [unwired: 9 in]
  n8 = register-events(error in=w10, w24) -> (reference out=w23:refnum<event-registration>, error out=w9:errorcluster)  [unwired: 1 in]
  n9 = call "XY Graph TipStrip Event Registration.vi"("error in (no error)"=w9, "XY Graph Refnum"=w5) -> ("error out"=w8:errorcluster, "Event Registration Refnum"=w14:refnum<event-registration>)  [unwired: 7 in, 1 out]
  n10 = call "Close Front Panel.vi"("error in (no error)"=w8, "VI in"=w7) -> ("VI out"=w6:refnum<vi>)  [unwired: 8 in, 1 out]
  n11 = call "AlliGator Queue.vi"() -> ("AlliGator Q"=w26:refnum<queue>)  [unwired: 8 in, 1 out]
  n12 = Bundle("Event Registration Refnum"=w23, "Event Registration Refnum"=w14) -> (w15:T3)  [unwired: 1 in]
  n13 = call "Get Notebook Queue.vi"() -> ("Notebook Queue"=w27:refnum<queue>)  [unwired: 9 in]
  n14 = while {
    tunnel: w27 -> [w39]
    tunnel: w26 -> [w37]
    tunnel: "AlliGator" ("Sender") -> [w35]
    tunnel: w6 -> [w33]
    tunnel: w15 -> [w32]
    tunnel: [w31] -> w22
    tunnel: [w30] -> w21
    tunnel: w5 -> [w28]
    stop <- w46 stop-if-true
    n15 = call "Busy Icon & Message Storage.vi"() -> ("Busy Icon Status (F = busy)"=w34:bool)  [unwired: 9 in, 2 out]
    n16 = event shown="[1] \"Lifetime & Other Parameters Graph\": Shortcut Menu Selection (User)" {
      selector: w32 -> [_ _ _ _ _ _ w176 w181 _]
      dyn-events: [_ _ _ _ _ _ w174 w179 _] -> w31
      timeout: _ -> [_ _ _ _ _ _ _ _ _]
      tunnel: [w50 w52 w100 _ w165 _ _ _ _] -> w40
      tunnel: [_ _ _ _ _ w168 _ _ _] -> w46
      tunnel: [_ w55 _ w121 _ _ _ _ _] -> w36
      tunnel: w34 -> [_ w61 _ _ _ _ _ _ _]
      tunnel: w35 -> [_ _ _ _ _ _ _ _ _]
      tunnel: w33 -> [w49 _ _ _ w167 _ _ _ _]
      tunnel: ["" ("Text") _ _ _ _ _ _ _ _] -> w29
      tunnel: w28 -> [_ w53 _ _ _ _ _ _ _]
      event Panel Close? {
        w48 = TRUE ("Pin Button")
        n17 = event-data() -> ()  [unwired: 1 in, 1 out]
        n18 = property on="Pin Button" class="Bool (strict)"("Value"=w48) -> (error out=w51:errorcluster)  [unwired: 2 in, 1 out]
        n19 = call "AlliGator Dock-Undock Subpanel Event.vi"("Error In"=w51, "Dock?"=w48, "VI in"=w49) -> ("Error Out"=w50:errorcluster)  [unwired: 8 in]
        n20 = event-data("Discard?"=w48) -> ()  [unwired: 1 in, 1 out]
      }
      event "Lifetime & Other Parameters Graph": Shortcut Menu Selection (User) {
        n21 = event-data() -> ("ItemPath"=w58:string, "CtlRef"=w57:refnum<vi>, "Coords"=w56:T8, "ItemTag"=w60:string)  [unwired: 1 in]
        n22 = Select(t=w60, s=w61, f="Busy") -> (s? t:f=w59:string)
        n23 = case shown="\"-----------------\"" w59 {
          selector: w59 -> [_ w64 _ _ _ _ _]
          tunnel: w57 -> [_ w66 _ _ _ w89 w96]
          tunnel: w56 -> [_ w65 _ _ _ w88 w95]
          tunnel: w58 -> [_ w63 _ _ _ _ _]
          tunnel: [_ w62 _ w76 w84 w91 w98] -> w55
          tunnel: w53 -> [_ _ _ w74 _ _ _]
          tunnel: [_ _ _ w71 _ _ _] -> w52
          frame "", "Busy" {
          }
          frame Default {
            n24 = Bundle By Name(cluster=T7 {"Item Tag"="", "XY Graph Refnum"=refnum, "Coords"={"Horizontal"=0, "Vertical"=0}, "Item Path"=""} ("XY Graph Event"), "Item Path"=w63, "XY Graph Refnum"=w66, "Coords"=w65, "Item Tag"=w64) -> (w69:T7)
            n25 = Bundle By Name(cluster=T5 {"AlliGator Q Event"=enum."Generic Graph:Generic XY Graph Event", "Data"=variant} ("element"), "Data"=w69) -> (w67:T5)
            n26 = Build Array(w67) -> (w62:T5[])
          }
          frame "-----------------" {
          }
          frame "New Plot" {
            w75 = T11 {"Multiplot XY Graph"=refnum, "Plot Name"="", "Plot Scales"={"X Scale"=0, "Y Scale"=0}, "Plot Interpolation"=enum."Use Previous Plot's Style", "Point Style"=enum."not defined", "Plot Color"=15781887, "Plot Metadata"=variant} ("New Plot Information")
            w78 = T5 {"AlliGator Q Event"=enum."Generic Graph:New Plot", "Data"=variant} ("Time-Gated Phasor Q Element")
            n27 = call "AlliGator Phasor Ratio Graph Ctrl Refnums.vi"() -> ("error out"=w71:errorcluster, "Phasor Ratio Graph Ctrl Refnums"=w73:T15)  [unwired: 10 in]
            n28 = Unbundle By Name(w73) -> ("Phasor Ratio Graph"=w72:refnum<vi>)
            n29 = Bundle By Name(cluster=w75, "Multiplot XY Graph"=w72, "Plot Name"="Phasor Ratio") -> (w82:T11)
            n30 = Bundle By Name(cluster=w75, "Multiplot XY Graph"=w74, "Plot Name"="Lifetime") -> (w79:T11)
            n31 = Bundle By Name(cluster=w78, "Data"=w82) -> (w83:T5)
            n32 = Bundle By Name(cluster=w78, "Data"=w79) -> (w77:T5)
            n33 = Build Array(w83, w77) -> (w76:T5[])
          }
          frame "Plot Decay Shifts" {
            n34 = Build Array(T5 {"AlliGator Q Event"=enum."Lifetime:Plot Decay Shifts", "Data"=variant} ("element")) -> (w84:T5[])
          }
          frame "Compute Sliced Mean, SDV and CV Plots" {
            n35 = Bundle By Name(cluster=T9 {"Multiplot XY Graph"=refnum, "Mouse Coordinates"={"Horizontal"=0, "Vertical"=0}} ("Mouse Click Event Data"), "Multiplot XY Graph"=w89, "Mouse Coordinates"=w88) -> (w86:T9)
            n36 = Bundle By Name(cluster=T5 {"AlliGator Q Event"=enum."Lifetime:Compute Sliced Mean, SDV and CV Plots", "Data"=variant} ("element"), "Data"=w86) -> (w90:T5)
            n37 = Build Array(w90) -> (w91:T5[])
          }
          frame "Plot Histogram" {
            n38 = Bundle By Name(cluster=T9 {"Multiplot XY Graph"=refnum, "Mouse Coordinates"={"Horizontal"=0, "Vertical"=0}} ("Mouse Click Event Data"), "Multiplot XY Graph"=w96, "Mouse Coordinates"=w95) -> (w93:T9)
            n39 = Bundle By Name(cluster=T5 {"AlliGator Q Event"=enum."Lifetime:Plot Histogram", "Data"=variant} ("element"), "Data"=w93) -> (w97:T5)
            n40 = Build Array(w97) -> (w98:T5[])
          }
        }
      }
      event "Lifetime & Other Parameters Graph": Shortcut Menu Activation? {
        n41 = event-data() -> ("CtlRef"=w102:refnum<vi>, "MenuRef"=w101:refnum<k9>)  [unwired: 1 in]
        n42 = call "XY Graph Check-Uncheck Menu Items.vi"("Menu in"=w101, "XY Graph Refnum"=w102) -> ("Error Out (dup)"=w111:errorcluster, "Menu out"=w106:refnum<k9>, "XY Graph Refnum dup"=w104:T10)  [unwired: 6 in, 1 out]
        n43 = call "XY Graph Get Label.vi"("XYGraph"=w104) -> ("Graph Label"=w103:string)  [unwired: 8 in]
        n44 = case shown="\"\", Default" w103 {
          tunnel: w111 -> [w112 w118]
          tunnel: [w112 w117] -> w107
          tunnel: w106 -> [w113 w116]
          tunnel: [w113 w115] -> w105
          frame "", Default {
          }
          frame "Decay Graph" {
            n45 = call "AlliGator Decay Graph Get-Set Process Plot Target.vi"("Get (F)/Set"=FALSE, "Error In"=w118, "Menu"=w116) -> ("Error Out (dup)"=w117:errorcluster, "Menu"=w115:refnum<k9>)  [unwired: 6 in, 1 out]
          }
        }
        n46 = call "AlliGator Add Python Functions to Object Menu.vi"("error in (no error)"=w107, "Menu in"=w105, "Object Refnum"=w104) -> ("error out"=w110:errorcluster, "Menu out"=w109:refnum<k9>, "Object Refnum dup"=w108:refnum<vi>)  [unwired: 6 in]
        n47 = call "AlliGator Grayed out Menu Items.vi"("error in (no error)"=w110, "Menu in"=w109, "Object Refnum"=w108) -> ("error out"=w100:errorcluster)  [unwired: 7 in, 1 out]
        n48 = event-data() -> ()  [unwired: 2 in, 1 out]
      }
      event "Lifetime & Other Parameters Graph": event #0x4e {
        n49 = event-data() -> ("ItemTag"=w122:string, "CtlRef"=w123:refnum<vi>, "Coords"=w120:T8, "ItemPath"=w119:string)  [unwired: 1 in]
        n50 = case shown="\"CURS_FREE\", \"CURS_MULTI\", \"CURS_SINGLE\"" w122 {
          selector: w122 -> [w128 _ _ _ _ _]
          tunnel: w123 -> [w127 w133 w139 _ w152 w159]
          tunnel: [w124 w135 w140 w149 w153 w160] -> w121
          tunnel: w120 -> [w126 _ _ _ w151 w158]
          tunnel: w119 -> [w125 _ _ _ _ _]
          frame "", Default {
            n51 = Bundle By Name(cluster=T7 {"Item Tag"="", "XY Graph Refnum"=refnum, "Coords"={"Horizontal"=0, "Vertical"=0}, "Item Path"=""} ("XY Graph Event"), "Item Tag"=w128, "XY Graph Refnum"=w127, "Coords"=w126, "Item Path"=w125) -> (w131:T7)
            n52 = Bundle By Name(cluster=T5 {"AlliGator Q Event"=enum."Generic Graph:Generic XY Graph Event", "Data"=variant} ("element"), "Data"=w131) -> (w129:T5)
            n53 = Build Array(w129) -> (w124:T5[])
          }
          frame "CURS_FREE", "CURS_MULTI", "CURS_SINGLE" {
            n54 = Bundle By Name(cluster=T5 {"AlliGator Q Event"=enum."Generic Graph:Set Last Cursor Style", "Data"=variant} ("AlliGator Actions"), "Data"=w133) -> (w134:T5)
            n55 = Build Array(w134) -> (w135:T5[])
          }
          frame "New Plot" {
            w141 = T11 {"Multiplot XY Graph"=refnum, "Plot Name"="", "Plot Scales"={"X Scale"=0, "Y Scale"=0}, "Plot Interpolation"=enum."Use Previous Plot's Style", "Point Style"=enum."not defined", "Plot Color"=15781887, "Plot Metadata"=variant} ("New Plot Information")
            w143 = T5 {"AlliGator Q Event"=enum."Generic Graph:New Plot", "Data"=variant} ("Time-Gated Phasor Q Element")
            n56 = call "AlliGator Phasor Ratio Graph Ctrl Refnums.vi"() -> ("Phasor Ratio Graph Ctrl Refnums"=w138:T15)  [unwired: 10 in, 1 out]
            n57 = Unbundle By Name(w138) -> ("Phasor Ratio Graph"=w137:refnum<vi>)
            n58 = Bundle By Name(cluster=w141, "Multiplot XY Graph"=w137, "Plot Name"="Phasor Ratio") -> (w147:T11)
            n59 = Bundle By Name(cluster=w141, "Multiplot XY Graph"=w139, "Plot Name"="Lifetime") -> (w144:T11)
            n60 = Bundle By Name(cluster=w143, "Data"=w147) -> (w148:T5)
            n61 = Bundle By Name(cluster=w143, "Data"=w144) -> (w142:T5)
            n62 = Build Array(w148, w142) -> (w140:T5[])
          }
          frame "Plot Decay Shifts" {
            n63 = Build Array(T5 {"AlliGator Q Event"=enum."Lifetime:Plot Decay Shifts", "Data"=variant} ("element")) -> (w149:T5[])
          }
          frame "Compute Sliced Mean, SDV and CV Plots" {
            n64 = Bundle By Name(cluster=T9 {"Multiplot XY Graph"=refnum, "Mouse Coordinates"={"Horizontal"=0, "Vertical"=0}} ("Mouse Click Event Data"), "Multiplot XY Graph"=w152, "Mouse Coordinates"=w151) -> (w157:T9)
            n65 = Bundle By Name(cluster=T5 {"AlliGator Q Event"=enum."Lifetime:Compute Sliced Mean, SDV and CV Plots", "Data"=variant} ("element"), "Data"=w157) -> (w155:T5)
            n66 = Build Array(w155) -> (w153:T5[])
          }
          frame "Plot Histogram" {
            n67 = Bundle By Name(cluster=T9 {"Multiplot XY Graph"=refnum, "Mouse Coordinates"={"Horizontal"=0, "Vertical"=0}} ("Mouse Click Event Data"), "Multiplot XY Graph"=w159, "Mouse Coordinates"=w158) -> (w164:T9)
            n68 = Bundle By Name(cluster=T5 {"AlliGator Q Event"=enum."Lifetime:Plot Histogram", "Data"=variant} ("element"), "Data"=w164) -> (w162:T5)
            n69 = Build Array(w162) -> (w160:T5[])
          }
        }
      }
      event "Pin Button": Value Change {
        n70 = event-data() -> ("NewVal"=w166:bool)  [unwired: 1 in]
        n71 = call "AlliGator Dock-Undock Subpanel Event.vi"("Dock?"=w166, "VI in"=w167) -> ("Error Out"=w165:errorcluster)  [unwired: 9 in]
      }
      event User Event {
        n72 = event-data() -> ("subpanel"=w170:string, "event"=w169:string)  [unwired: 1 in]
        n73 = case shown="\"AlliGator\"" w170 {
          tunnel: w169 -> [_ w172]
          tunnel: [_ w171] -> w168
          frame "False", Default {
          }
          frame "AlliGator" {
            n74 = case shown="\"False\", Default" w172 {
              tunnel: [_ TRUE] -> w171
              frame "False", Default {
              }
              frame "quit" {
              }
            }
          }
        }
      }
      event Mouse Enter {
        n75 = event-data() -> ("CtlRef"=w175:refnum<vi>)  [unwired: 1 in]
        n76 = Unbundle By Name(w176) -> ("Event Registration Refnum"=w178:refnum<event-registration>)
        n77 = call "XY Graph Tipstrip Mouse Enter.vi"("Event Registration Refnum"=w178, "XY Graph Refnum"=w175) -> ("Event Registration Refnum"=w177:refnum<event-registration>)  [unwired: 8 in, 1 out]
        n78 = Bundle By Name(cluster=w176, "Event Registration Refnum"=w177) -> (w174:T3)
      }
      event Mouse Leave {
        n79 = event-data() -> ("CtlRef"=w180:refnum<vi>)  [unwired: 1 in]
        n80 = Unbundle By Name(w181) -> ("Event Registration Refnum"=w182:refnum<event-registration>)
        n81 = call "XY Graph Tipstrip Mouse Leave.vi"("Event Registration Refnum"=w182, "XY Graph Refnum"=w180) -> ("Event Registration Refnum"=w183:refnum<event-registration>)  [unwired: 8 in, 1 out]
        n82 = Bundle By Name(cluster=w181, "Event Registration Refnum"=w183) -> (w179:T3)
      }
      event Mouse Move {
        n83 = event-data() -> ("CtlRef"=w186:refnum<vi>, "Coords"=w185:T8)  [unwired: 1 in]
        n84 = control-ref of="Lifetime & Other Parameters Graph TipStrip"() -> (w184:refnum<vi>)
        n85 = call "XY Graph Set Plot TipStrip.vi"("TipStrip Refnum"=w184, "Max Length (200)"=300, "Coords"=w185, "XY Graph Refnum"=w186) -> ()  [unwired: 5 in, 3 out]
      }
    }
    n86 = call "AlliGator Settings Storage.vi"("AlliGator Settings List"=AlliGator_Settings_List."Miscellaneous:Verbose Error Mode") -> ("Variant Data out"=w45:variant)  [unwired: 9 in, 1 out]
    n87 = call-poly "Variant to Data.vi"("Variant"=w45) -> ("Value"=w38:bool)  [unwired: 8 in]
    n88 = call "Send Message to Notebook.vi"("Error In"=w40, "Text"=w29, "Notebook Queue"=w39) -> ("Error Out"=w42:errorcluster, "Notebook Queue"=w41:refnum<queue>)  [unwired: 5 in]
    n89 = call "Light Theme Message Style.vi"() -> ()  [unwired: 1 out]
    n90 = call "AlliGator Queue Non Empty Events.vi"("Actions"=w36, "AlliGator Q"=w37) -> ()  [unwired: 9 in, 1 out]
    n91 = call "Send Error to Notebook.vi"("error in (no error)"=w42, "Verbose Error Messages (T)"=w38, "State Machine Case Error Source"="Lifetime Graph", "Notebook Q"=w41) -> ("Error Out"=w30:errorcluster)  [unwired: 7 in]
  }
  n92 = call "Tiny Clear Error.vi"("Error In"=w21) -> ("no Error Out"=w20:errorcluster)  [unwired: 8 in]
  n93 = Unregister For Events(event registration refnum=w22) -> (error out=w12:errorcluster)  [unwired: 1 in]
  n94 = invoke class="VI" method="FP.Close"(reference=w6, error in=w20) -> (error out=w13:errorcluster)  [unwired: 1 in, 2 out]
  n95 = Merge Errors(w13, w12) -> (w11:errorcluster)
  n96 = call "Tiny Clear Error.vi"("Error In"=w11) -> ()  [unwired: 8 in, 1 out]
